vi "PicoScope2000Settings.vi"(1 "Unit Info":T1, 4 "Channel B Settings":T2={"Enabled"=FALSE, "Coupling"=1, "Range"=6} {"Range" items=["20 mV"=1, "50 mV"=2, "100 mV"=3, "200 mV"=4, "500 mV"=5, "1 V"=6, "2 V"=7, "5 V"=8, "10 V"=9, "20 V"=10]; "Coupling" items=["AC", "DC"]}, 5 "Channel A Settings":T2={"Enabled"=FALSE, "Coupling"=1, "Range"=6} {"Range" items=["20 mV"=1, "50 mV"=2, "100 mV"=3, "200 mV"=4, "500 mV"=5, "1 V"=6, "2 V"=7, "5 V"=8, "10 V"=9, "20 V"=10]; "Coupling" items=["AC", "DC"]}, 6 "Trigger Settings":T3={"Trigger Enabled"=FALSE, "Trigger Source"=enum."Channel A", "Trigger Threshold (V)"=0.0, "Trigger Direction"=0, "Trigger Delay (%)"=0, "Auto Trigger Time (ms)"=1000} {"Trigger Direction" items=["Rising", "Falling"]; "Trigger Threshold (V)" format="%.3f"}, 7 "Max ADC value":i16=32767, 8 "handle in":i16, 9 "error in":errorcluster) -> (0 "Enabled Array":i16[](array[numeric]), 2 "handle out":i16, 3 "error out":errorcluster)   [LabVIEW 2010]
doc: "This VI is used to set up the oscilloscope. The inputs are clusters for setting channel and simple trigger settings. Advanced triggers can be set up using PicoScope3000aAdvancedTriggerSettings.vi"
uses:
  ps2000.dll
  PicoScope2000AnalogChannelSettings.ctl
panel:
  out "Numeric 4":i16
  in  "Channel D range":i16=10
  in  "Channel D dc":i16
  in  "Channel D enabled":i16
  out "Numeric 3":i16
  in  "Channel C range":i16=2
  in  "Channel C dc":i16
  in  "Channel C enabled":i16
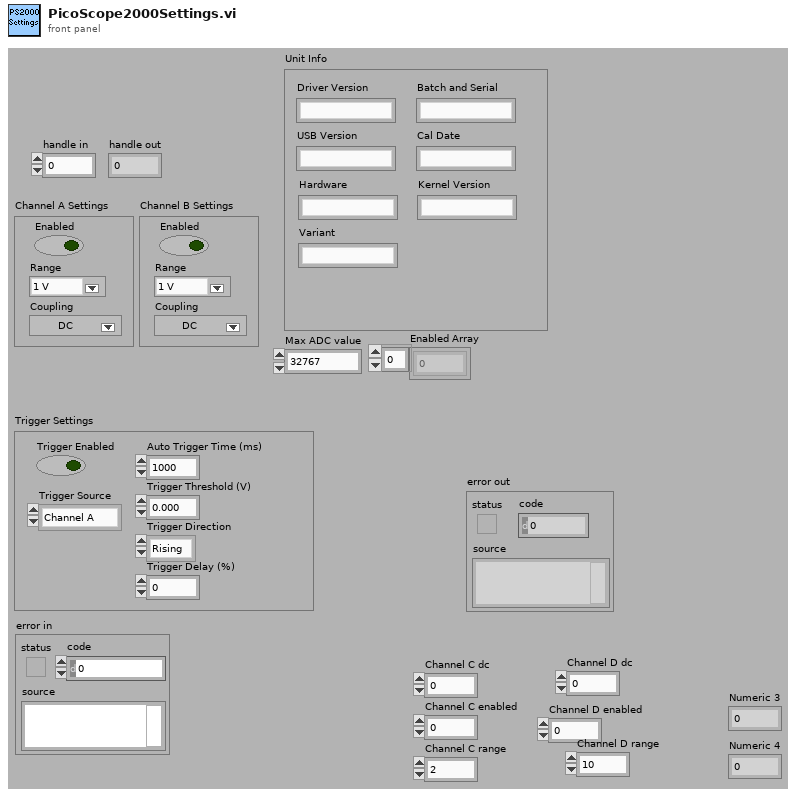
[diagram p1: front panel]
types:
  T1 = cluster{"Driver Version":string, "USB Version":string, "Hardware":string, "Variant":string, "Batch and Serial":string, "Cal Date":string, "Kernel Version":string}
  T2 = typedef "PicoScope2000AnalogChannelSettings.ctl" = cluster{"Enabled":bool, "Coupling":i16, "Range":u16}
  T3 = cluster{"Trigger Enabled":bool, "Trigger Source":enum16{"Channel A", "Channel B"}, "Trigger Threshold (V)":dbl, "Trigger Direction":i16, "Trigger Delay (%)":i16, "Auto Trigger Time (ms)":i16}
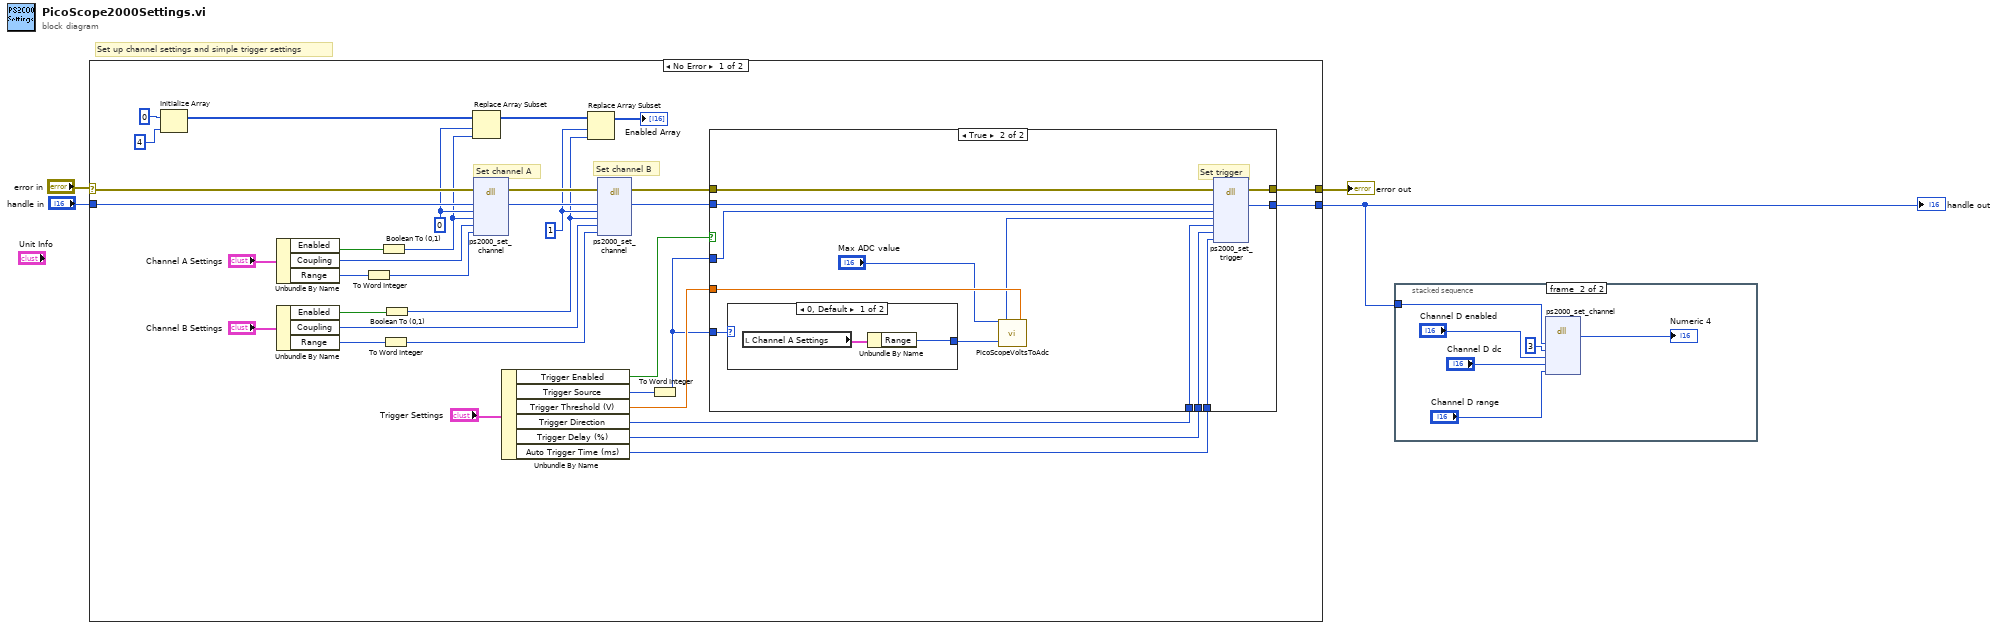
[diagram p0: block diagram]
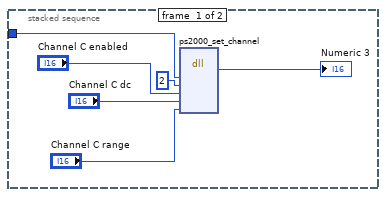
[diagram p2: hidden frame]
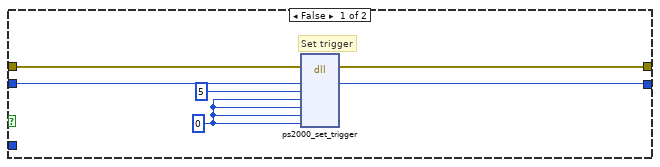
[diagram p3: hidden frame]
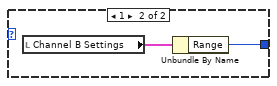
[diagram p4: hidden frame]
diagram:
  # "Set up channel settings and simple trigger settings"
  n1 = case shown="No Error" "error in" {
    selector: "error in" -> [w36 w64]
    tunnel: "handle in" -> [w35 w63]
    tunnel: [w25 w63] -> w1
    tunnel: [w26 w64] -> w2
    frame No Error {
      w7 = i16 1 ("channel")
      w10 = i16 0 ("channel")
      # "Set channel B"
      # "Set channel A"
      n2 = Initialize Array(i16 0 ("element"), 4 ("dimension size")) -> (w11:i16[])
      n3 = Unbundle By Name("Channel A Settings") -> ("Enabled"=w34:bool, "Coupling"=w33:i16, "Range"=w32:u16)
      n4 = Unbundle By Name("Channel B Settings") -> ("Enabled"=w29:bool, "Coupling"=w28:i16, "Range"=w16:u16)
      n5 = To Word Integer(number=w32) -> (16bit integer=w15:i16)
      n6 = Boolean To (0,1)(Boolean=w34) -> (0, 1=w9:i16)
      n7 = To Word Integer(number=w16) -> (16bit integer=w14:i16)
      n8 = Boolean To (0,1)(Boolean=w29) -> (0, 1=w6:i16)
      n9 = Replace Array Subset(array=w11, new element=w9, index=w10) -> (w8:i16[])
      n10 = dll-call lib="PS2000.dll" fn="ps2000_set_channel"(error in=w36, "handle"=w35, "channel"=w10, "enabled"=w9, "dc"=w33, "range"=w15) -> (error out=w30:errorcluster, "handle"=w31:i16)  [unwired: 7 in, 1 out]
      n11 = Unbundle By Name("Trigger Settings") -> ("Trigger Enabled"=w23:bool, "Trigger Source"=w18:enum16{"Channel A", "Channel B"}, "Trigger Threshold (V)"=w19:dbl, "Trigger Direction"=w22:i16, "Trigger Delay (%)"=w21:i16, "Auto Trigger Time (ms)"=w20:i16)
      n12 = Replace Array Subset(array=w8, new element=w6, index=w7) -> (→"Enabled Array":i16[])
      n13 = dll-call lib="PS2000.dll" fn="ps2000_set_channel"(error in=w30, "handle"=w31, "channel"=w7, "enabled"=w6, "dc"=w28, "range"=w14) -> (error out=w24:errorcluster, "handle"=w27:i16)  [unwired: 7 in, 1 out]
      n14 = To Word Integer(number=w18) -> (16bit integer=w17:i16)
      n15 = case shown="True" w23 {
        tunnel: w27 -> [w45 w58]
        tunnel: [w42 w57] -> w25
        tunnel: [w41 w56] -> w26
        tunnel: w24 -> [w40 w55]
        tunnel: w17 -> [_ w54]
        tunnel: w22 -> [_ w46]
        tunnel: w21 -> [_ w53]
        tunnel: w20 -> [_ w52]
        tunnel: w19 -> [_ w49]
        tunnel: w17 -> [_ w51]
        frame False {
          w43 = i16 0 ("auto_trigger_ms")
          # "Set trigger"
          n16 = dll-call lib="ps2000.dll" fn="ps2000_set_trigger"(error in=w40, "handle"=w45, "source"=i16 5, "threshold"=w43, "direction"=w43, "delay"=w43, "auto_trigger_ms"=w43) -> (error out=w41:errorcluster, "handle"=w42:i16)  [unwired: 8 in, 1 out]
        }
        frame True {
          # "Set trigger"
          n17 = case shown="0, Default" w51 {
            tunnel: [w59 w61] -> w50
            frame 0, Default {
              n18 = local read "Channel A Settings"() -> (w60:T2)
              n19 = Unbundle By Name(w60) -> ("Range"=w59:u16)
            }
            frame 1 {
              n20 = local read "Channel B Settings"() -> (w62:T2)
              n21 = Unbundle By Name(w62) -> ("Range"=w61:u16)
            }
          }
          n22 = call "PicoScopeVoltsToAdc.vi"("Max_adc"="Max ADC value", "Volts"=w49, "Range Index"=w50) -> ("ADC count"=w47:i16)
          n23 = dll-call lib="PS2000.dll" fn="ps2000_set_trigger"(error in=w55, "handle"=w58, "source"=w54, "threshold"=w47, "direction"=w46, "delay"=w53, "auto_trigger_ms"=w52) -> (error out=w56:errorcluster, "handle"=w57:i16)  [unwired: 8 in, 1 out]
        }
      }
    }
    frame Error {
    }
  }
  "handle out" <- w1
  "error out" <- w2
  n24 = stacked-sequence {
    tunnel: w1 -> [w65 w71]
    frame #0 {
      n25 = dll-call lib="PS2000.dll" fn="ps2000_set_channel" label="ps2000_set_channel_C"("handle"=w65, "channel"=i16 2, "enabled"="Channel C enabled", "dc"="Channel C dc", "range"="Channel C range") -> ("return type"=→"Numeric 3":i16)  [unwired: 8 in, 2 out]
    }
    frame #1 {
      n26 = dll-call lib="PS2000.dll" fn="ps2000_set_channel" label="ps2000_set_channel_D"("handle"=w71, "channel"=i16 3, "enabled"="Channel D enabled", "dc"="Channel D dc", "range"="Channel D range") -> ("return type"=→"Numeric 4":i16)  [unwired: 8 in, 2 out]
    }
  }
